vi "Find and Rename Libraries.vi"(0 "Owned Items[]":refnum<vi>[](array[refnum]), 2 "Private Data.Application Ref":refnum<vi>, 5 "new name":string, 7 "name to replace":string, 11 "error in":errorcluster) -> (15 "error out":errorcluster)   [LabVIEW 2022 SP3, in "Springboard TLB`.lvlib"]
uses:
  Springboard TLB`.lvlib
  <vilib>/regexp/Match Regular Expression.xnode
panel:
  out "Array 2":string[](array[string])
  out "Array":string[](array[string])
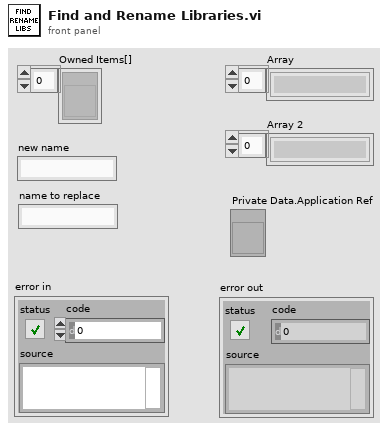
[diagram p1: front panel]
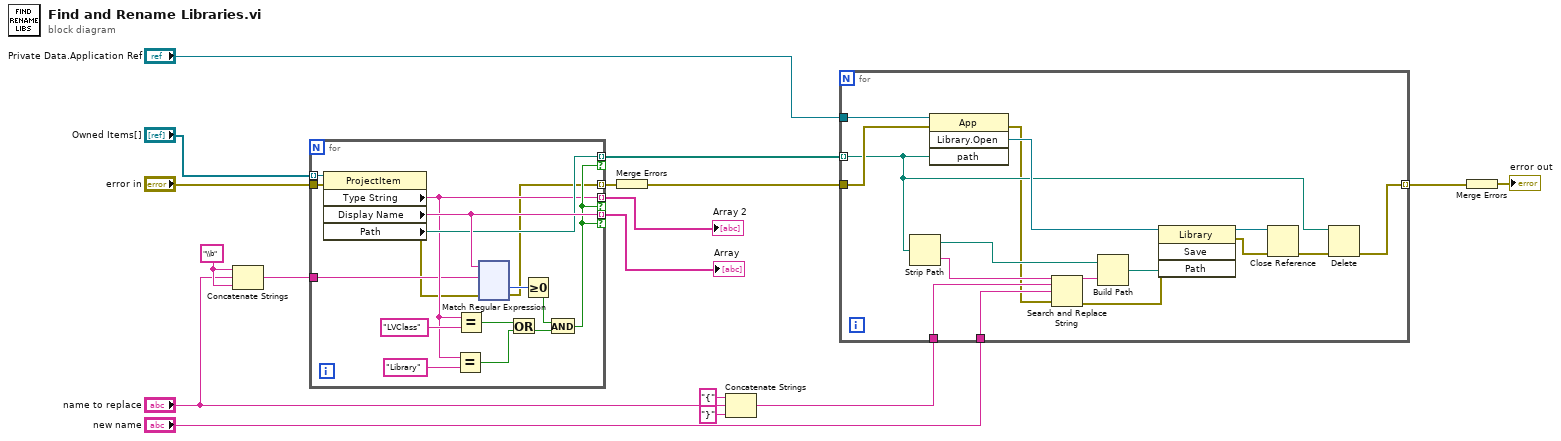
[diagram p0: block diagram]
diagram:
  w6 = "\\b" ("string")
  n1 = Concatenate Strings(w6, "name to replace", w6) -> (w7:string)
  n2 = for {
    tunnel: "Owned Items[]" -> [w33] mode=indexing
    tunnel: [w22] -> w13 mode=indexing if=w29
    tunnel: [w31] -> w14 mode=indexing if=w29
    tunnel: [w26] -> w8 mode=indexing if=w29
    tunnel: [w18] -> w16 mode=indexing
    tunnel: "error in" -> [w28]
    tunnel: w7 -> [w20]
    n3 = property class="ProjectItem"(reference=w33, error in=w28) -> (error out=w19:errorcluster, "Type String"=w22:string, "Display Name"=w31:string, "Path"=w26:path)  [unwired: 1 out]
    n4 = Equal?(x=w22, y="Library") -> (x = y?=w21:bool)
    n5 = Equal?(x=w22, y="LVClass") -> (x = y?=w24:bool)
    n6 = xnode "Match Regular Expression"("input string"=w31, "regular expression"=w20, "error in"=w19) -> ("offset past match"=w30:i32, "error out"=w18:errorcluster)  [unwired: 3 in, 3 out]
    n7 = Or(x=w24, y=w21) -> (x .or. y?=w25:bool)
    n8 = Greater Or Equal To 0?(x=w30) -> (x >= 0?=w27:bool)
    n9 = And(x=w27, y=w25) -> (x .and. y?=w29:bool)
  }
  "Array" <- w14
  "Array 2" <- w13
  n10 = Merge Errors(w16) -> (w17:errorcluster)
  n11 = Concatenate Strings("{" ("string"), "name to replace", "}" ("string")) -> (w2:string)
  n12 = for {
    tunnel: "Private Data.Application Ref" -> [w166]
    tunnel: w8 -> [w154] mode=indexing
    tunnel: w17 -> [w165]
    tunnel: [w155] -> w11 mode=indexing
    tunnel: "new name" -> [w157]
    tunnel: w2 -> [w153]
    n13 = Strip Path(path=w154) -> (stripped path=w158:path, name=w160:string)
    n14 = invoke class="App" method="Library.Open"(reference=w166, error in=w165, "path"=w154) -> (error out=w152:errorcluster, "Open Library"=w164:refnum<vi>)  [unwired: 1 in, 2 out]
    n15 = Search and Replace String(input string=w160, search string=w153, replace string=w157, error in=w152) -> (result string=w159:string, error out=w151:errorcluster)  [unwired: 4 in, 2 out]
    n16 = Build Path(base path=w158, name or relative path=w159) -> (appended path=w156:path)
    n17 = invoke class="Library" method="Save"(reference=w164, error in=w151, "Path"=w156) -> (reference out=w162:refnum<vi>, error out=w163:errorcluster)  [unwired: 1 in, 2 out]
    n18 = Close Reference(reference=w162, error in (no error)=w163) -> (error out=w161:errorcluster)
    n19 = Delete(path (use dialog)=w154, error in=w161) -> (error out=w155:errorcluster)  [unwired: 3 in, 2 out]
  }
  n20 = Merge Errors(w11) -> (→"error out":errorcluster)
